vi "FuncVI-NotifSend.vi"(5 "InstanceRef":T2, 9 "arg list":T1[](array[typedef]) {"num" format="%.2f"}) -> (0 "error out":bool, 3 "result":T1 {"num" format="%.2f"})   [LabVIEW 2021]
doc: "::: CalcExpress Toolkit :::\nCopyright (c) 2000-2026 Konstantin Shifershteyn. All rights reserved."
uses:
  cetypes.llb/CalcExpress Function Argument Info.ctl
  cetypes.llb/CalcExpress Instance RefNum.ctl
panel:
  in  "max arg num":i32=2
  in  "min arg num":i32=1
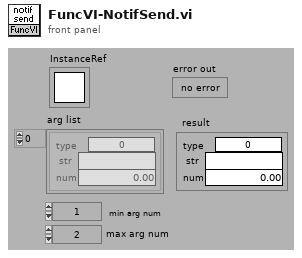
[diagram p1: front panel]
types:
  T1 = typedef "CalcExpress Function Argument Info.ctl" = cluster{"type":u32, "str":string, "num":dbl}
  T2 = typedef "CalcExpress Instance RefNum.ctl" = refnum<k1>
  T3 = enum32{"String", "DBL Number", "identifier", "1D Array of DBL", "2D Array of DBL", "CDB Number", "1D Array of CDB", "2D Array of CDB", "1D Array of String", "2D Array of String", "Unknown data type"}
  T4 = cluster{"data type":enum32{"String", "DBL Number", "identifier", "1D Array of DBL", "2D Array of DBL", "CDB Number", "1D Array of CDB", "2D Array of CDB", "1D Array of String", "2D Array of String", "Unknown data type"}, string, dbl}
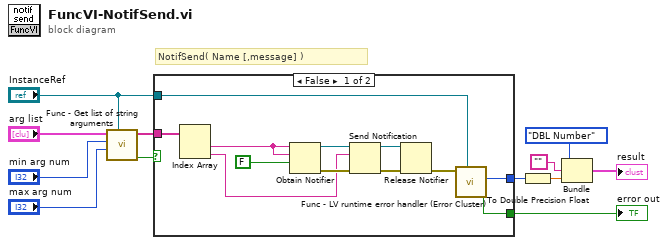
[diagram p0: block diagram]
diagram:
  # "NotifSend( Name [,message] )"
  n1 = call "Func - Get list of string arguments.vi"("InstanceRef"="InstanceRef", "max arg num"="max arg num", "min arg num"="min arg num", "arg list"="arg list") -> ("error out"=w4:bool, "val list"=w11:string[])  [unwired: 4 in]
  n2 = case shown="False" w4 {
    selector: w4 -> [_ w25]
    tunnel: w11 -> [w24 _]
    tunnel: "InstanceRef" -> [w21 _]
    tunnel: [w19 _] -> w5
    tunnel: [w20 w25] -> w3
    frame False {
      n3 = Index Array(array=w24) -> (element #1=w14:string, element #2=w18:string)  [unwired: 2 in]
      n4 = Obtain Notifier(name (unnamed)=w14, notification data type=w14, create if not found? (T)=FALSE) -> (notifier out=w23:refnum<notifier>, error out=w22:errorcluster)  [unwired: 1 in, 1 out]
      n5 = Send Notification(notification=w18, notifier=w23, error in (no error)=w22) -> (notifier out=w17:refnum<notifier>, error out=w16:errorcluster)
      n6 = Release Notifier(notifier=w17, error in (no error)=w16) -> (error out=w15:errorcluster)  [unwired: 1 in, 2 out]
      n7 = call "Func - LV runtime error handler (Error Cluster).vi"("InstanceRef"=w21, "LabVIEW error"=w15) -> ("error out"=w20:bool, "LV error code"=w19:i32)  [unwired: 4 in, 2 out]
    }
    frame True {
    }
  }
  "error out" <- w3
  n8 = To Double Precision Float(number=w5) -> (double precision float=w10:dbl)
  n9 = Bundle("data type"=T3."DBL Number", "", w10) -> (→"result":T4)  [unwired: 1 in]
